vi "Highscore_Save.vi"(0 "Table":cluster{"Score":i32, "Name":string}[](array[cluster]), 11 "error in":errorcluster) -> (15 "error out":errorcluster)   [LabVIEW 2020, in "GH_Engine.lvlib"]
doc: "Writes the highscore list to Resourcesòta\\highscores.txt (Score;Name per line)."
uses:
  GH_Engine.lvlib
  Level/GH_Level.lvlib
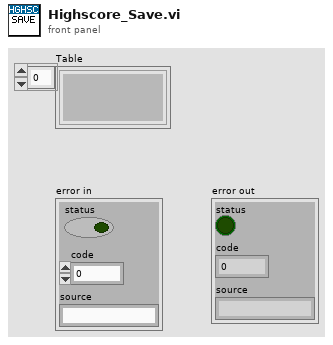
[diagram p1: front panel]
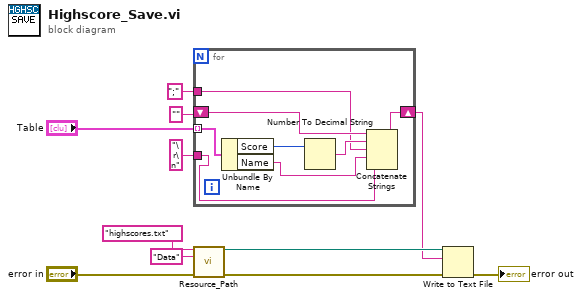
[diagram p0: block diagram]
diagram:
  n1 = for {
    tunnel: "Table" -> [w12] mode=indexing
    tunnel: ";" -> [w13]
    tunnel: "\r\n" -> [w14]
    shift-right: [w16] -> w6
    shift-left: "" -> [w15]
    n2 = Unbundle By Name(w12) -> ("Score"=w17:i32, "Name"=w18:string)
    n3 = Number To Decimal String(number=w17) -> (decimal integer string=w19:string)  [unwired: 1 in]
    n4 = Concatenate Strings(w15, w19, w13, w18, w14) -> (w16:string)
  }
  n5 = call "Resource_Path.vi"("File name"="highscores.txt", "Subfolder"="Data", "error in"="error in") -> ("Path"=w9:path, "error out"=w10:errorcluster)  [unwired: 11 in]
  n6 = Write to Text File(file (use dialog)=w9, text=w6, error in=w10) -> (error out=→"error out":errorcluster)  [unwired: 1 in, 2 out]
